vi "VIH HelpGen - FILE - Get Type.vi"(8 "error in":errorcluster, 11 "File Path":path) -> (0 "error out":errorcluster, 2 "File Type":T1, 3 "dup File Path":path)   [LabVIEW 2014]
doc: "::: VI Helpeks :::\nCopyright (c) 2000-2026 Konstantin Shifershteyn. All rights reserved."
uses:
  _VIH HelpGen - Palette.llb/VIH HelpGen Typedef - Palette - Item Type Enum.ctl
  <vilib>/Utility/lvfile.llb/FT_FileTypes.ctl
  <vilib>/Utility/lvfile.llb/NI_FileType.lvlib
panel:
  # "VI Helpeks\nCopyright (c) 2012-2026 Konstantin Shifershteyn"
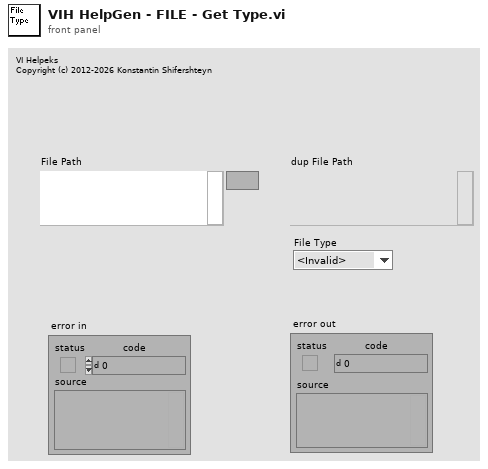
[diagram p1: front panel]
types:
  T1 = typedef "VIH HelpGen Typedef - Palette - Item Type Enum.ctl" = enum32{"<Invalid>", "<unknown>", "VI", "Menu", "LV Func", "Express VI", "Poly VI", "CTL", "HTML"}
  T2 = typedef "NI_FileType.lvlib/FT_FileTypes.ctl" = enum32{"Invalid file/path", "Unknown type", "Instrument", "Control", "Polymorphic VI", "Project", "Library", "LVClass", "XControl", "XNode", "CIN", "Run-time menu", "Palette menu", "LLB", "Shortcut", "Directory", "Class Private Data Control", "Statechart", "MathScript .m file", "Ladder Diagram", "LVLibp"}
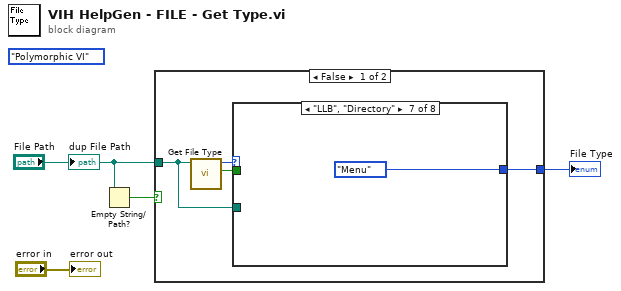
[diagram p0: block diagram]
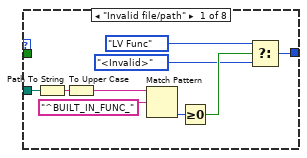
[diagram p2: hidden frame]
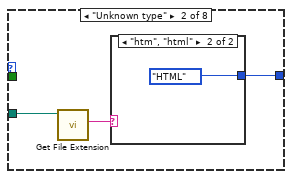
[diagram p3: hidden frame]
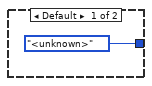
[diagram p4: hidden frame]
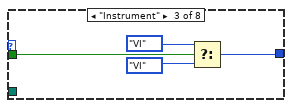
[diagram p5: hidden frame]
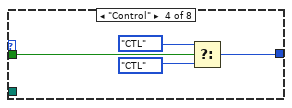
[diagram p6: hidden frame]
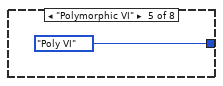
[diagram p7: hidden frame]
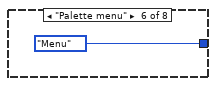
[diagram p8: hidden frame]
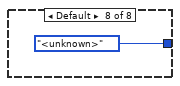
[diagram p9: hidden frame]
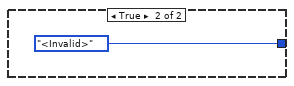
[diagram p10: hidden frame]
diagram:
  (unwired) FT_FileTypes."Polymorphic VI" ("file type")
  n1 = Empty String/Path?(string/path="File Path") -> (empty?=w4:bool)
  n2 = case shown="False" w4 {
    tunnel: "File Path" -> [w5 _]
    tunnel: [w6 VIH_HelpGen_Typedef_-_Palette_-_Item_Type_Enum."<Invalid>" ("Item Type")] -> w3
    frame False {
      n3 = call <vilib>:"Get File Type.vi"("path"=w5) -> ("is template?"=w7:bool, "file type"=w8:T2)  [unwired: 8 in, 1 out]
      n4 = case shown="\"LLB\", \"Directory\"" w8 {
        tunnel: w7 -> [_ _ w26 w30 _ _ _ _]
        tunnel: [w11 w20 w25 w29 VIH_HelpGen_Typedef_-_Palette_-_Item_Type_Enum."Poly VI" ("Item Type") VIH_HelpGen_Typedef_-_Palette_-_Item_Type_Enum."Menu" ("Item Type") VIH_HelpGen_Typedef_-_Palette_-_Item_Type_Enum."Menu" ("Item Type") VIH_HelpGen_Typedef_-_Palette_-_Item_Type_Enum."<unknown>" ("Item Type")] -> w6
        tunnel: w5 -> [w17 w19 _ _ _ _ _ _]
        frame "Invalid file/path" {
          n5 = Path To String(path=w17) -> (string=w16:string)
          n6 = To Upper Case(1:w16) -> (0:w15:string)
          n7 = Match Pattern(string=w15, regular expression="^BUILT_IN_FUNC_") -> (offset past match=w13:i32)  [unwired: 1 in, 3 out]
          n8 = Greater Or Equal To 0?(x=w13) -> (x >= 0?=w12:bool)
          n9 = Select(t=VIH_HelpGen_Typedef_-_Palette_-_Item_Type_Enum."LV Func" ("Item Type"), s=w12, f=VIH_HelpGen_Typedef_-_Palette_-_Item_Type_Enum."<Invalid>") -> (s? t:f=w11:T1)
        }
        frame "Unknown type" {
          n10 = call <vilib>:"Get File Extension.vi"("file"=w19) -> ("lowercase file extension"=w18:string)  [unwired: 7 in, 3 out]
          n11 = case shown="\"htm\", \"html\"" w18 {
            tunnel: [VIH_HelpGen_Typedef_-_Palette_-_Item_Type_Enum."<unknown>" ("Item Type") VIH_HelpGen_Typedef_-_Palette_-_Item_Type_Enum."HTML" ("Item Type")] -> w20
            frame Default {
            }
            frame "htm", "html" {
            }
          }
        }
        frame "Instrument" {
          n12 = Select(t=VIH_HelpGen_Typedef_-_Palette_-_Item_Type_Enum."VI" ("Item Type"), s=w26, f=VIH_HelpGen_Typedef_-_Palette_-_Item_Type_Enum."VI" ("Item Type")) -> (s? t:f=w25:T1)
        }
        frame "Control" {
          n13 = Select(t=VIH_HelpGen_Typedef_-_Palette_-_Item_Type_Enum."CTL" ("Item Type"), s=w30, f=VIH_HelpGen_Typedef_-_Palette_-_Item_Type_Enum."CTL" ("Item Type")) -> (s? t:f=w29:T1)
        }
        frame "Polymorphic VI" {
        }
        frame "Palette menu" {
        }
        frame "LLB", "Directory" {
        }
        frame Default {
        }
      }
    }
    frame True {
    }
  }
  "File Type" <- w3
  "error out" <- "error in"
  "dup File Path" <- "File Path"
